vi "Make Protection Signal.vi"(11 "Node Ptr":T1=18446744073709551615 format="%.0x") -> ()   [LabVIEW 2025, in "Protection and Counter Addon System Explorer.lvlib"]
uses:
  Protection and Counter Addon System Explorer.lvlib
  Addon Shared/SubVIs/GUID Lookup.vi
  Addon Shared/Protection and Counter Addon Shared.lvlib
  SubModules/Frame-Protection-Support/Source/System Explorer/Protection and Counter Support System Explorer.lvlib
  SubModules/Frame-Protection-Support/Source/Shared/Types/Protection Type.ctl
  SubModules/Frame-Protection-Support/Source/Shared/Protection and Counter Support Shared.lvlib
  SubModules/Frame-Protection-Support/Source/System Explorer/Types/Switch Protection Signal Settings.ctl
  SubModules/Frame-Protection-Support/Source/System Explorer/Types/Switch GUID Settings.ctl
  <vilib>/NI VeriStand/Custom Device API/Custom Device Item Ref.ctl
  <vilib>/NI VeriStand/Custom Device API/Custom Device API.lvlib
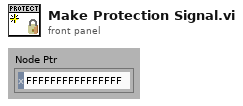
[diagram p1: front panel]
types:
  T1 = typedef "Custom Device API.lvlib/Custom Device Item Ref.ctl" = u64
  T2 = typedef "Switch GUID Settings.ctl" = cluster{"Incoming Page":string, "Protection Value":string, "Protected Signal":string, "Signal Page":string, "Invalid Count Channel":string, "Counter Value Channel":string}
  T3 = typedef "Protection and Counter Support System Explorer.lvlib/Switch Protection Signal Settings.ctl" = cluster{"Default Protection Type":T4, "Include All Channels":bool}
  T4 = typedef "Protection and Counter Support Shared.lvlib/Protection Type.ctl" = enum16{"Arb ID + Bytes Checksum with Inversion", "Arb ID + Bytes CRC with Inversion", "Reversed Raw Signal Checksum with Inversion", "Concatenated Two's Compliment"}
  T5 = typedef "Protection and Counter Addon Shared.lvlib/XNET Settings.ctl" = cluster{"Database":refnum<k21>, "Cluster":refnum<k21>, "Port":string, "Baud rate [Bd]":u64, "Termination":u32, "CAN I/O Mode":u32, "FD Baud rate [Bd]":u64, "Priority":i32, "Use Legacy":bool, "FD ISO Mode":u32, "Default Max Counter Value":dbl, "Default Protect Type":T4, "Include All Channels":bool}
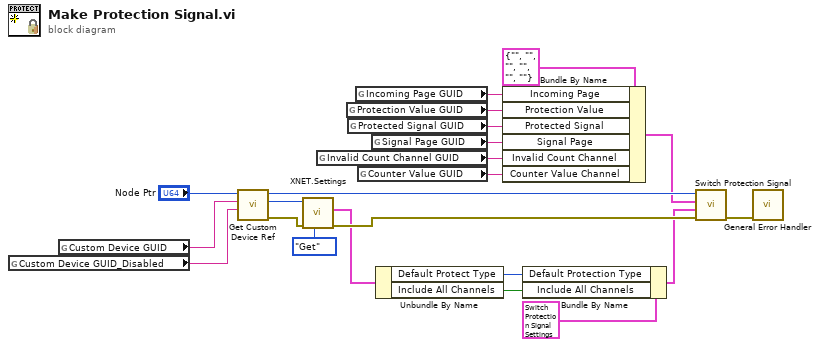
[diagram p0: block diagram]
diagram:
  n1 = global read "GUID Lookup.vi" "Custom Device GUID_Disabled"() -> (w18:string)
  n2 = global read "GUID Lookup.vi" "Custom Device GUID"() -> (w17:string)
  n3 = call "Get Custom Device Ref.vi"("Custom Device GUID_Disabled"=w18, "Custom Device GUID"=w17, "Section Ptr"="Node Ptr") -> ("error out"=w20:errorcluster, "Custom Device Ref"=w19:T1, "Section Ref out"=w15:T1)  [unwired: 6 in]
  n4 = call "XNET.Settings.vi"("Action"=enum8{"Get", "Set"}."Get", "error in (no error)"=w20, "Parent Ref in"=w19) -> ("error out"=w14:errorcluster, "XNET Settings"=w13:T5)  [unwired: 6 in, 1 out]
  n5 = global read "GUID Lookup.vi" "Invalid Count Channel GUID"() -> (w6:string)
  n6 = global read "GUID Lookup.vi" "Protection Value GUID"() -> (w4:string)
  n7 = global read "GUID Lookup.vi" "Protected Signal GUID"() -> (w8:string)
  n8 = global read "GUID Lookup.vi" "Incoming Page GUID"() -> (w9:string)
  n9 = global read "GUID Lookup.vi" "Counter Value GUID"() -> (w5:string)
  n10 = global read "GUID Lookup.vi" "Signal Page GUID"() -> (w7:string)
  n11 = Unbundle By Name(w13) -> ("Default Protect Type"=w11:T4, "Include All Channels"=w10:bool)
  n12 = Bundle By Name(cluster=T2 {"Incoming Page"="", "Protection Value"="", "Protected Signal"="", "Signal Page"="", "Invalid Count Channel"="", "Counter Value Channel"=""} ("GUIDs"), "Incoming Page"=w9, "Protection Value"=w4, "Protected Signal"=w8, "Signal Page"=w7, "Invalid Count Channel"=w6, "Counter Value Channel"=w5) -> (w1:T2)
  n13 = Bundle By Name(cluster=T3 {"Default Protection Type"=enum."Arb ID + Bytes Checksum with Inversion", "Include All Channels"=FALSE} ("Settings"), "Default Protection Type"=w11, "Include All Channels"=w10) -> (w2:T3)
  n14 = call "Switch Protection Signal.vi"("error in (no error)"=w14, "Settings"=w2, "GUIDs"=w1, "Node Ptr"=w15) -> ("error out"=w22:errorcluster)  [unwired: 7 in]
  n15 = call <vilib>:"General Error Handler.vi"("error in (no error)"=w22) -> ()  [unwired: 10 in, 5 out]
